vi "test 9401 DIO Scan Mode Loop Back.vi"(8 "error in (no error)":errorcluster, 11 "TestCase in":refnum<class "Scan Engine EtherCAT System Tests.lvclass">) -> (0 "error out":errorcluster, 3 "TestCase out":refnum<class "Scan Engine EtherCAT System Tests.lvclass">)   [LabVIEW 2020, in "Scan Engine EtherCAT System Tests.lvclass"]
uses:
  Scan Engine EtherCAT System Tests.lvclass
  C:/Program Files (x86)/National Instruments/LabVIEW 2020/vi.lib/NI/VeriStand Custom Device Testing Tools/VeriStandTestCase/VeriStandTestCase.lvclass
  <vilib>/addons/_JKI Toolkits/VI Tester/TestCase.llb/TestCase.lvclass
  <vilib>/NI/VeriStand Custom Device Testing Tools/VeriStandTestCase/VeriStandTestCase.lvclass
  System Explorer/SEECD System Explorer.lvlib
  C:/Program Files (x86)/National Instruments/LabVIEW 2020/vi.lib/addons/_JKI Toolkits/VI Tester/TestCase.llb/TestCase.lvclass
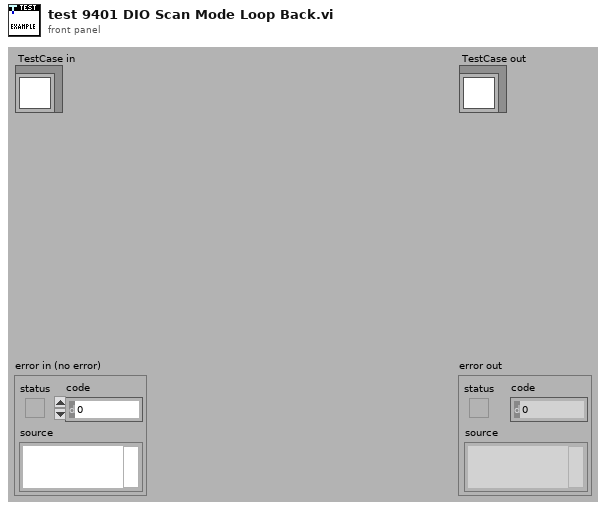
[diagram p1: front panel]
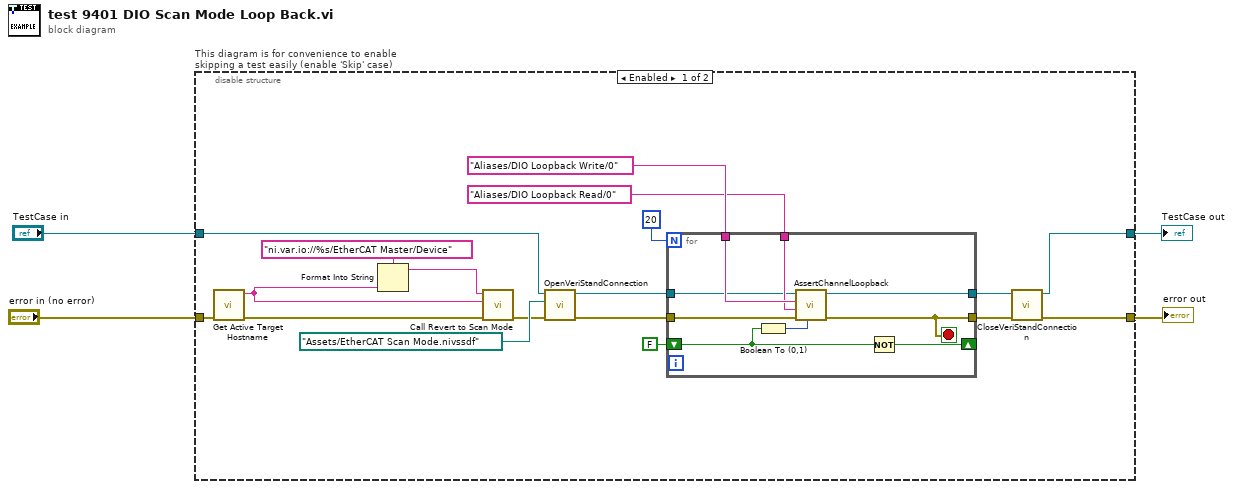
[diagram p0: block diagram]
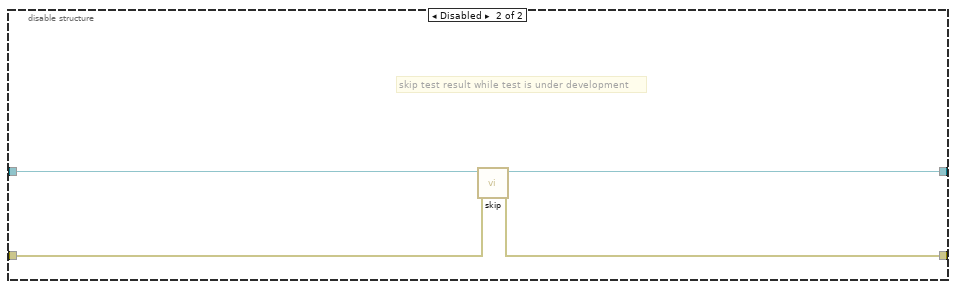
[diagram p2: hidden frame]
diagram:
  n1 = disable-structure "This diagram is for convenience to enable skipping a test easily (enable 'Skip' case)" shown="Enabled" {
    disable-tunnel: "TestCase in" -> [w16 w35]
    disable-tunnel: [w12 w33] -> w1
    disable-tunnel: [w13 w34] -> w3
    disable-tunnel: "error in (no error)" -> [w8 w32]
    frame Enabled {
      n2 = call "Get Active Target Hostname.vi"("error in"=w8) -> ("error out"=w7:errorcluster, "IP Address / Hostname"=w6:string)  [unwired: 9 in]
      n3 = Format Into String(format string="ni.var.io://%s/EtherCAT Master/Device", w6) -> (resulting string=w5:string)  [unwired: 2 in, 1 out]
      n4 = call "Call Revert to Scan Mode.vi"("error in"=w7, "Target IP Address"=w6, "Slave Ref"=w5) -> ("error out"=w10:errorcluster)  [unwired: 8 in]
      n5 = call-dynamic "OpenVeriStandConnection.vi"("error in (no error)"=w10, "System Definition File"=path "Assets/EtherCAT Scan Mode.nivssdf", "VeriStand Test Case in"=w16) -> ("error out"=w18:errorcluster, "VeriStand Test Case out"=w17:refnum<class "Scan Engine EtherCAT System Tests.lvclass">)  [unwired: 6 in, 1 out]
      n6 = for {
        N: 20 -> [_]
        tunnel: "Aliases/DIO Loopback Write/0" ("Channel") -> [w28]
        tunnel: [w26] -> w15
        tunnel: "Aliases/DIO Loopback Read/0" ("Channel") -> [w27]
        shift-right: [w31] -> _
        shift-left: FALSE -> [w30]
        tunnel: w18 -> [w29]
        tunnel: [w23] -> w14
        tunnel: w17 -> [w24]
        stop <- w26 stop-if-true
        n7 = Boolean To (0,1)(Boolean=w30) -> (0, 1=w25:i16)
        n8 = call <vilib>:"AssertChannelLoopback.vi"("Value"=w25, "error in (no error)"=w29, "Read Channel"=w27, "Write Channel"=w28, "VeriStand Test Case in"=w24) -> ("error out"=w26:errorcluster, "VeriStand Test Case out"=w23:refnum<class "Scan Engine EtherCAT System Tests.lvclass">)  [unwired: 5 in]
        n9 = Not(x=w30) -> (.not. x?=w31:bool)
      }
      n10 = call-dynamic "CloseVeriStandConnection.vi"("error in (no error)"=w15, "VeriStand Test Case in"=w14) -> ("error out"=w13:errorcluster, "VeriStand Test Case out"=w12:refnum<class "Scan Engine EtherCAT System Tests.lvclass">)  [unwired: 8 in]
    }
    frame Disabled {
      # "skip test result while test is under development"
      n11 = call <vilib>:"skip.vi"("error in (no error)"=w32, "TestCase in"=w35) -> ("error out"=w34:errorcluster, "TestCase out"=w33:refnum<class "Scan Engine EtherCAT System Tests.lvclass">)  [unwired: 8 in]
    }
  }
  "error out" <- w3
  "TestCase out" <- w1
